vi "Menu.Sequeunce.Execute.vi"(8 "error in (no error)":errorcluster, 9 "Coords":T1, 10 "ItemPath":string, 11 "State Variables":T2={"Aliases.All"=[], "Aliases.Outputs"=[], "UI.Sequence#ofColumns"=0, "SysDef.Path"=path "", "UI.SequenceRef"=refnum, "UI.StepInformationRef"=refnum, "UI.AbortRef"=refnum, "UI.GraphRef"=refnum, "UI.ViewRef"=refnum, "UI.IterationsRef"=refnum, "UI.IterationInformationRef"=refnum, "INI.Settings"={"Build Location"=path "C:/Simple Sequence Editor/SequenceRepo", "LoggingLocation"=path ""}, "NIVS.Workspace Event"=refnum, "UI.SkipChannel"=refnum, "NIVS.Launched?"=FALSE, "UI.DurationChannel"=refnum}) -> (0 "error out":errorcluster, 3 "State Variables out":T2={"Aliases.All"=[], "Aliases.Outputs"=[], "UI.Sequence#ofColumns"=0, "SysDef.Path"=path "", "UI.SequenceRef"=refnum, "UI.StepInformationRef"=refnum, "UI.AbortRef"=refnum, "UI.GraphRef"=refnum, "UI.ViewRef"=refnum, "UI.IterationsRef"=refnum, "UI.IterationInformationRef"=refnum, "INI.Settings"={"Build Location"=path "C:/Simple Sequence Editor/SequenceRepo", "LoggingLocation"=path ""}, "NIVS.Workspace Event"=refnum, "UI.SkipChannel"=refnum, "NIVS.Launched?"=FALSE, "UI.DurationChannel"=refnum})   [LabVIEW 2015, in "Simple Sequence Tools - Editor.lvlib"]
uses:
  Simple Sequence Tools - Editor.lvlib
  Types/Main.StateVariables.ctl
  Shared/Types/Channel.Properties.ctl
  Shared/Types/INI.Settings.ctl
  <vilib>/Utility/miscctls.llb/LVPoint32TypeDef.ctl
  <vilib>/Utility/miscctls.llb/LVBoundsTypeDef.ctl
  Shared/SubVIs/Main.Constants.vi
  Shared/Simple Sequence Tools - Shared.lvlib
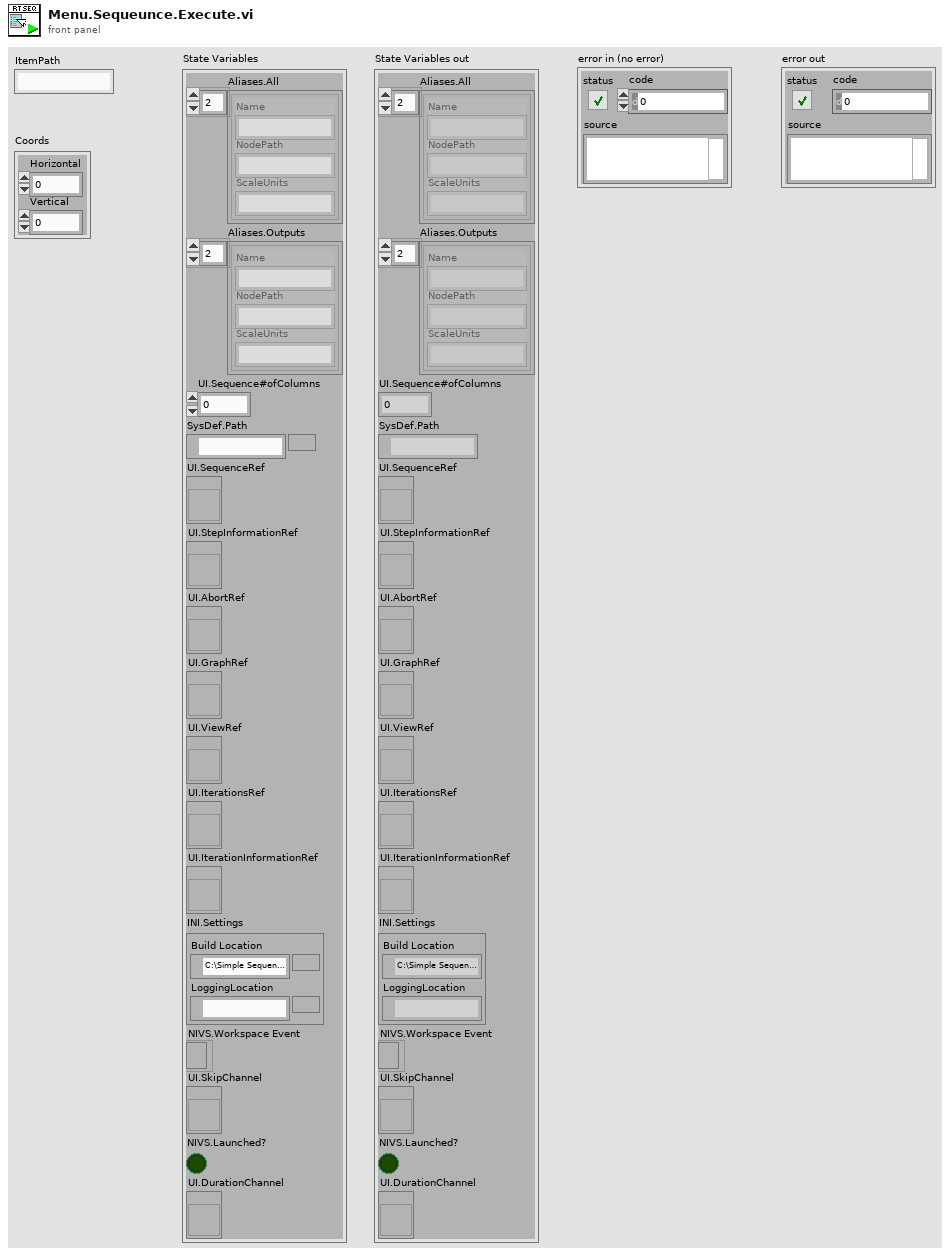
[diagram p1: front panel]
types:
  T1 = typedef "LVPoint32TypeDef.ctl" = cluster{"Horizontal":i32, "Vertical":i32}
  T2 = typedef "Simple Sequence Tools - Editor.lvlib/Main.StateVariables.ctl" = cluster{"Aliases.All":T3[], "Aliases.Outputs":T3[], "UI.Sequence#ofColumns":i32, "SysDef.Path":path, "UI.SequenceRef":refnum<vi>, "UI.StepInformationRef":refnum<vi>, "UI.AbortRef":refnum<vi>, "UI.GraphRef":refnum<vi>, "UI.ViewRef":refnum<vi>, "UI.IterationsRef":refnum<vi>, "UI.IterationInformationRef":refnum<vi>, "INI.Settings":T4, "NIVS.Workspace Event":refnum<event-registration>, "UI.SkipChannel":refnum<vi>, "NIVS.Launched?":bool, "UI.DurationChannel":refnum<vi>}
  T3 = typedef "Simple Sequence Tools - Shared.lvlib/Channel.Properties.ctl" = cluster{"Name":string, "NodePath":string, "ScaleUnits":string}
  T4 = typedef "Simple Sequence Tools - Shared.lvlib/INI.Settings.ctl" = cluster{"Build Location":path, "LoggingLocation":path}
  T5 = typedef "LVRowAndColumnTypeDef.ctl" = cluster{"Row":i32, "Column":i32}
  T6 = typedef "LVBoundsTypeDef.ctl" = cluster{"Width":u32, "Height":u32}
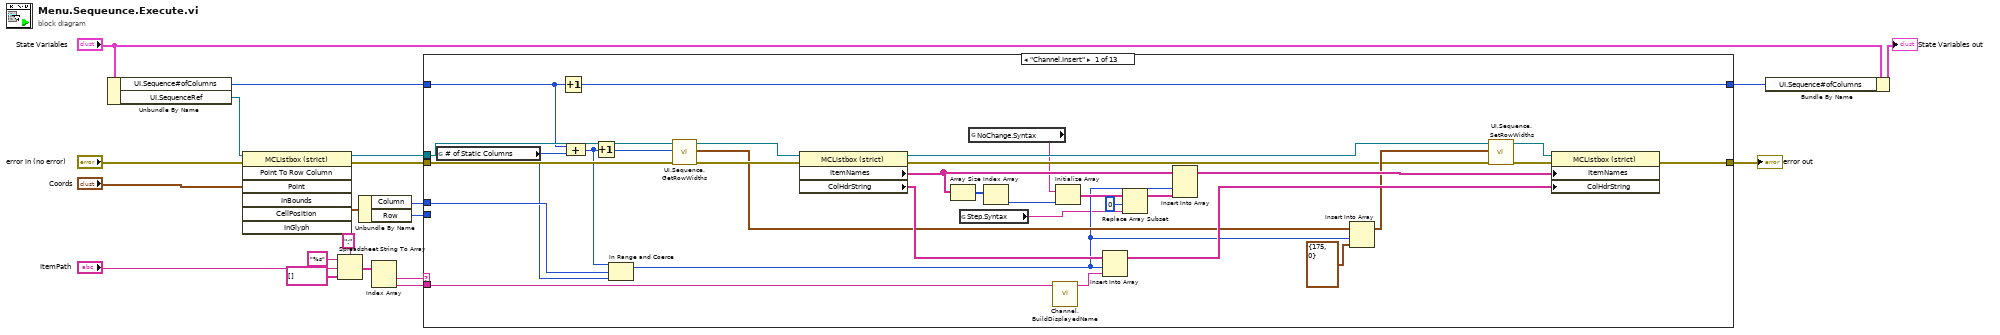
[diagram p0: block diagram]
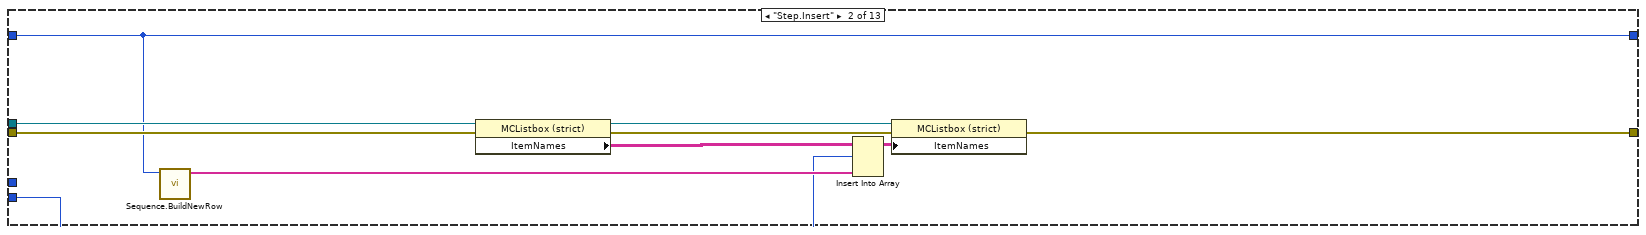
[diagram p2: hidden frame]
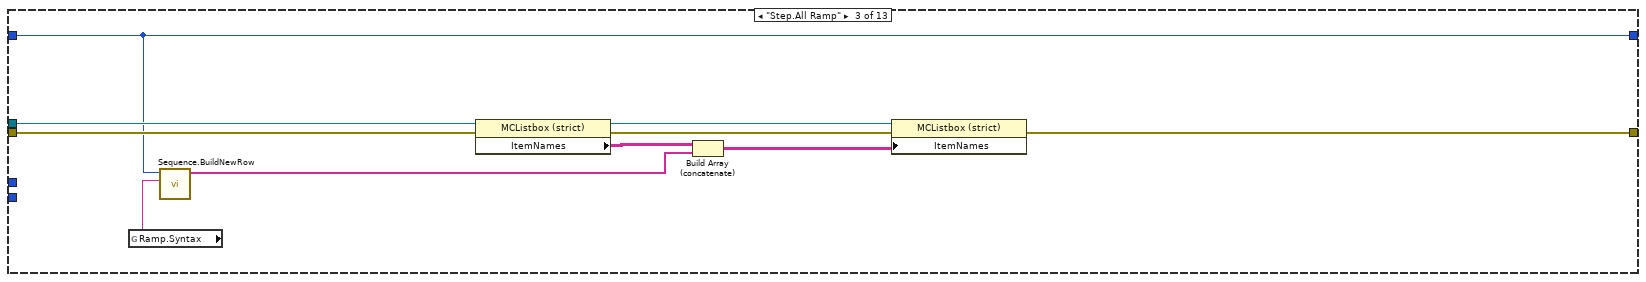
[diagram p3: hidden frame]
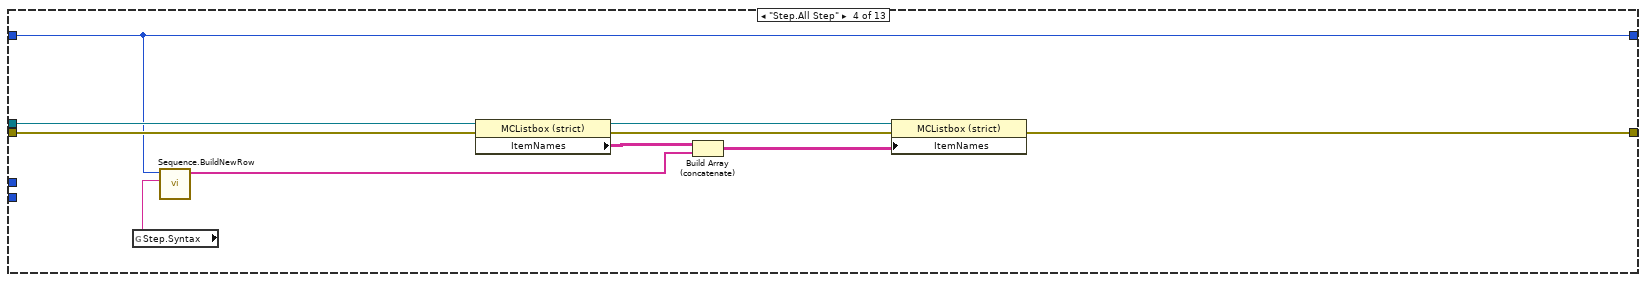
[diagram p4: hidden frame]
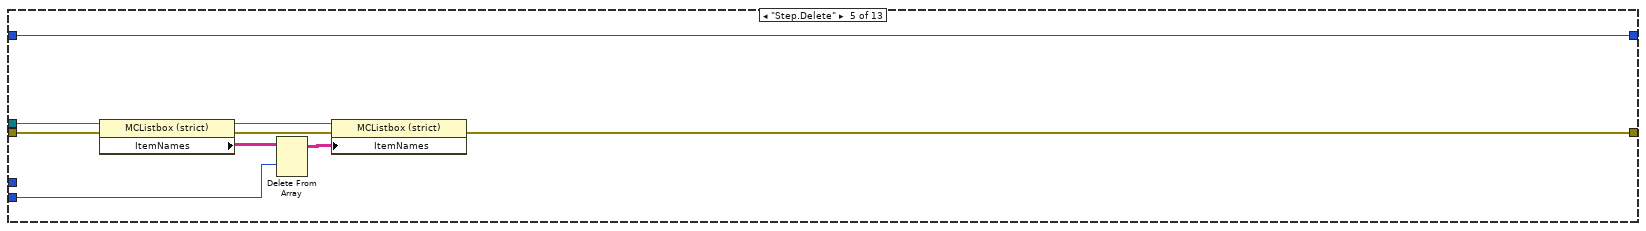
[diagram p5: hidden frame]
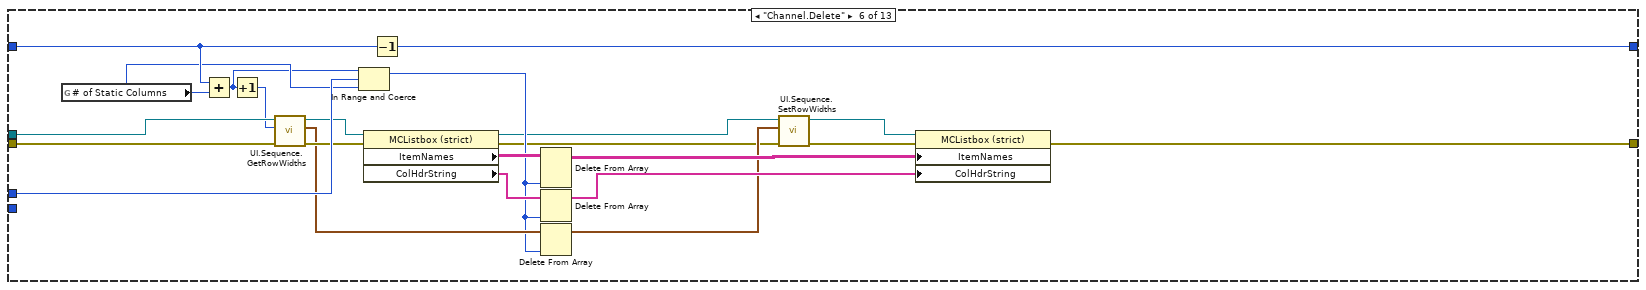
[diagram p6: hidden frame]
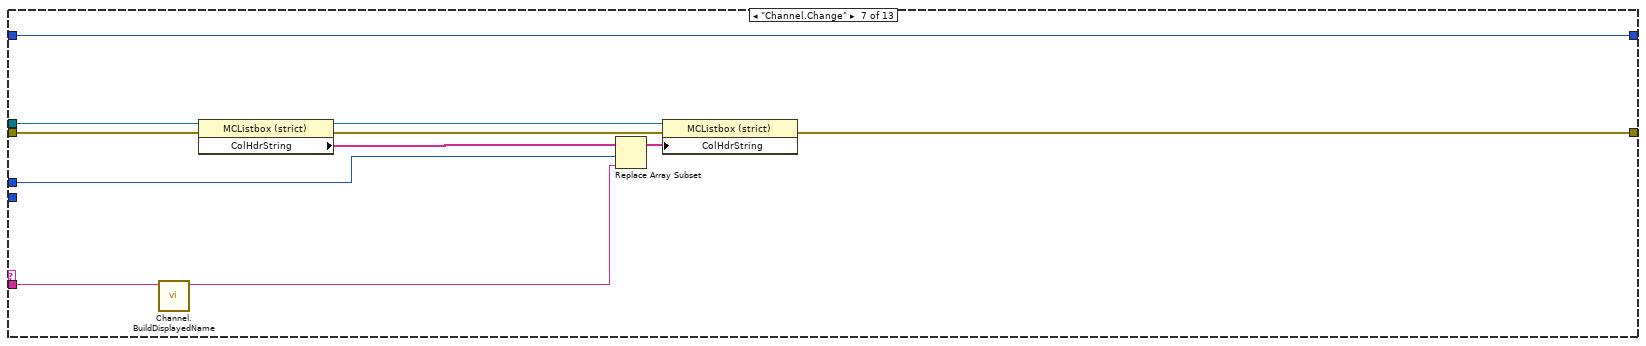
[diagram p7: hidden frame]
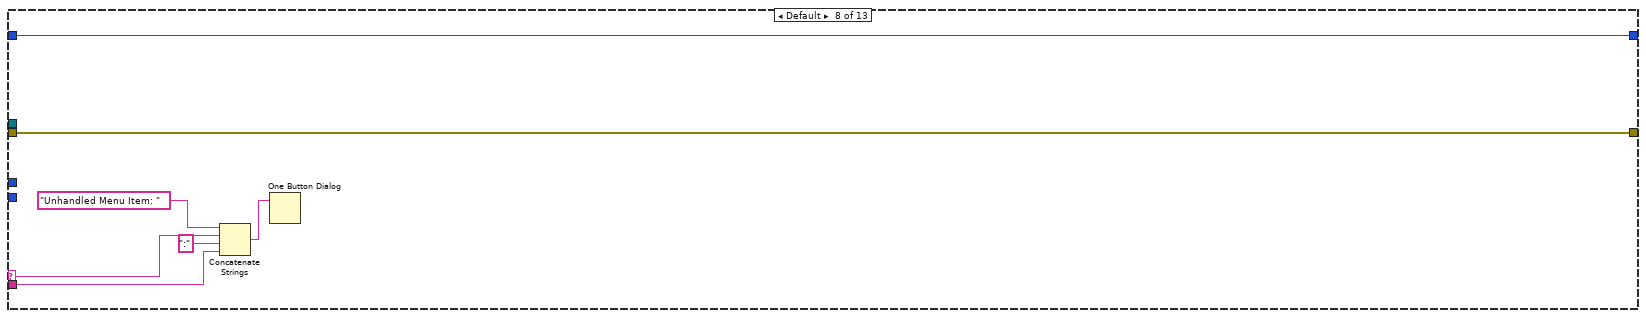
[diagram p8: hidden frame]
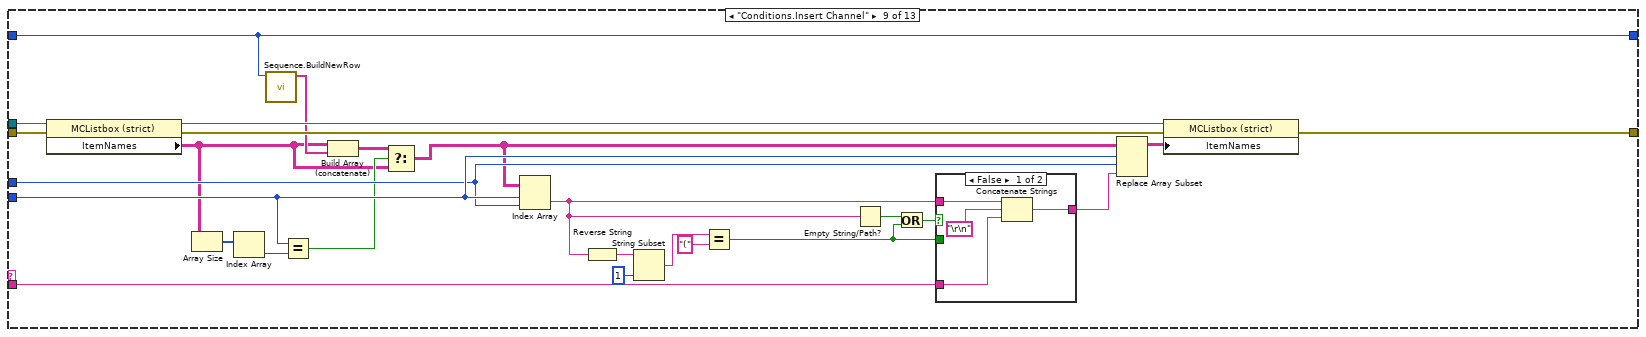
[diagram p9: hidden frame]
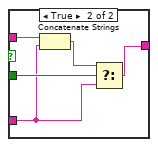
[diagram p10: hidden frame]
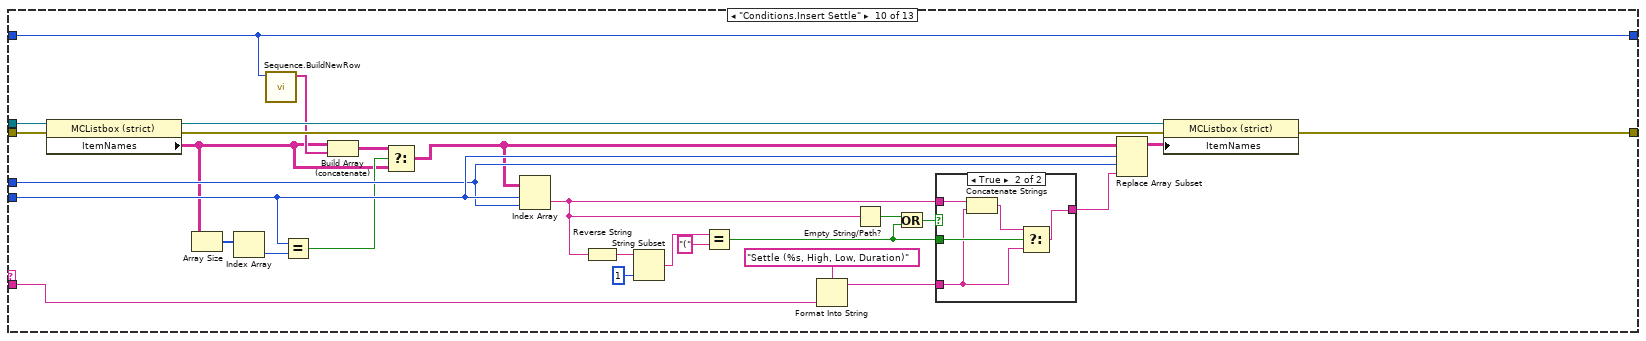
[diagram p11: hidden frame]
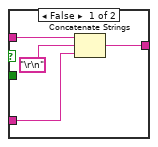
[diagram p12: hidden frame]
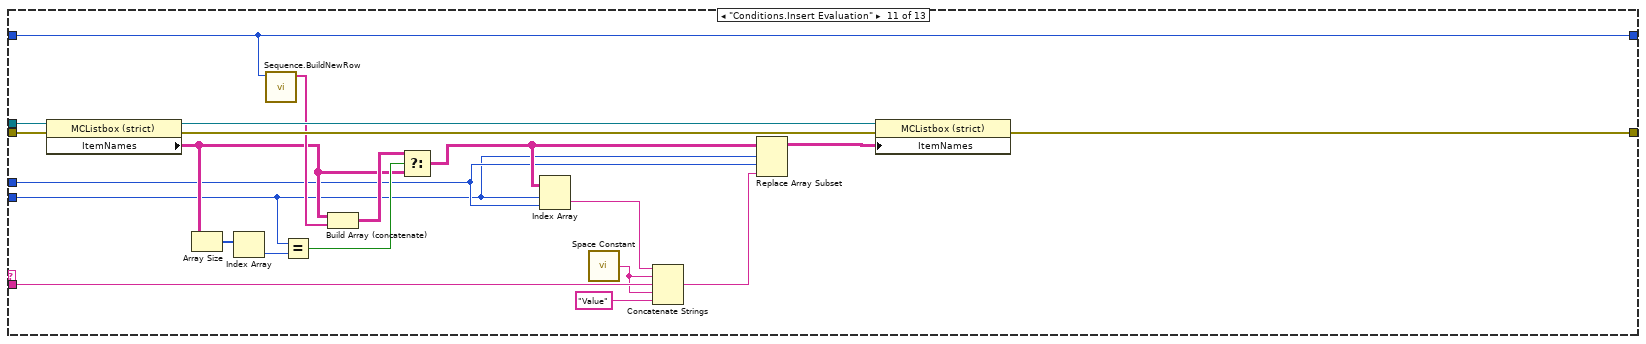
[diagram p13: hidden frame]
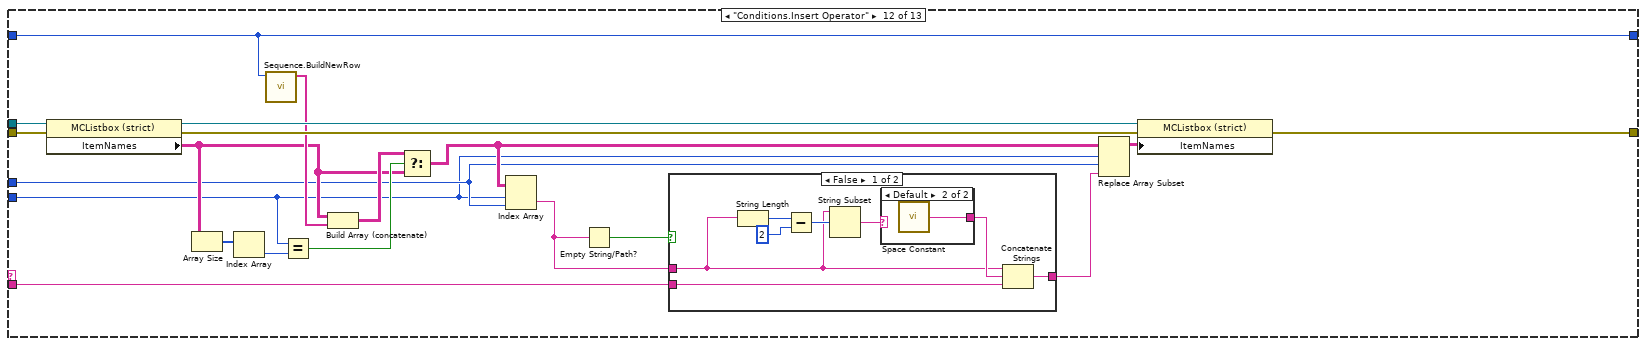
[diagram p14: hidden frame]
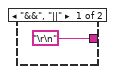
[diagram p15: hidden frame]
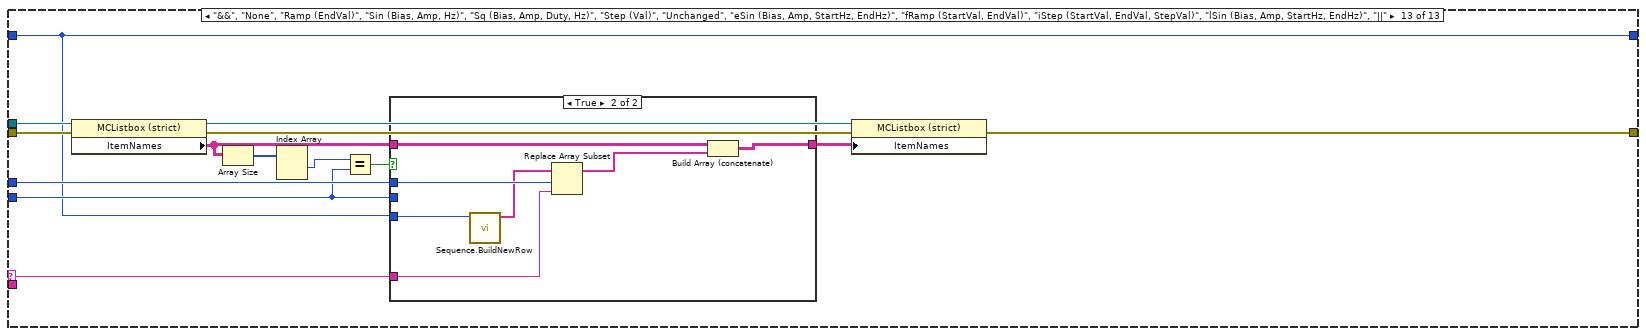
[diagram p17: hidden frame]
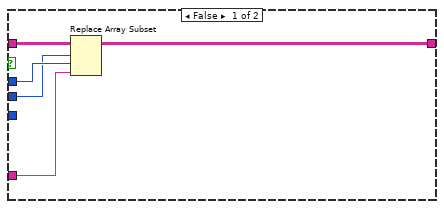
[diagram p18: hidden frame]
diagram:
  n1 = Unbundle By Name("State Variables") -> ("UI.Sequence#ofColumns"=w11:i32, "UI.SequenceRef"=w8:refnum<vi>)
  n2 = invoke class="MCListbox (strict)" method="Point To Row Column"(reference=w8, error in="error in (no error)", "Point"="Coords") -> (reference out=w13:refnum<vi>, error out=w14:errorcluster, "CellPosition"=w10:T5)  [unwired: 4 in, 4 out]
  n3 = Spreadsheet String To Array(delimiter (Tab)=":", format string="%s", spreadsheet string="ItemPath", array type (2D Dbl)=string[] []) -> (array=w6:string[])
  n4 = Unbundle By Name(w10) -> ("Column"=w12:i32, "Row"=w1:i32)
  n5 = Index Array(array=w6) -> (element #1=w7:string, element #2=w15:string)  [unwired: 2 in]
  n6 = case shown="\"Channel.Insert\"" w7 {
    selector: w7 -> [_ _ _ _ _ _ _ w129 _ _ _ _ w258]
    tunnel: w11 -> [w36 w53 w65 w75 w83 w100 w124 w131 w148 w186 w217 w237 w256]
    tunnel: w12 -> [w52 _ _ _ _ w113 w117 _ w142 w180 w207 w228 w264]
    tunnel: w13 -> [w38 w58 w68 w78 w87 w105 w118 _ w157 w194 w224 w244 w268]
    tunnel: w14 -> [w40 w59 w69 w79 w88 w107 w119 w130 w156 w193 w223 w243 w269]
    tunnel: w15 -> [w42 _ _ _ _ _ w115 w127 w152 w167 w219 w239 _]
    tunnel: [w24 w60 w70 w80 w89 w94 w116 w130 w154 w191 w221 w241 w257] -> w17
    tunnel: [w35 w53 w65 w75 w83 w112 w124 w131 w148 w186 w217 w237 w256] -> w20
    tunnel: w1 -> [_ w54 _ _ w84 _ _ _ w145 w183 w206 w227 w260]
    frame "Channel.Insert" {
      n7 = global read "Main.Constants.vi" "# of Static Columns"() -> (w22:u32)
      n8 = Increment(x=w36) -> (x+1=w35:i32)
      n9 = Compound Arithmetic op=ADD(w36, w22) -> (w21:u32)
      n10 = Increment(x=w21) -> (x+1=w30:u32)
      n11 = In Range and Coerce(upper limit=w21, x=w52, lower limit=w22) -> (coerced(x)=w32:u32)  [unwired: 1 out]
      n12 = call "UI.Sequence.GetRowWidths.vi"("error in (no error)"=w40, "Numeric"=w30, "UI.SequenceRef"=w38) -> ("error out"=w39:errorcluster, "Array"=w33:T6[], "UI.SequenceRef"=w37:refnum<vi>)  [unwired: 6 in]
      n13 = property class="MCListbox (strict)"(reference=w37, error in=w39) -> (reference out=w25:refnum<vi>, error out=w28:errorcluster, "ItemNames"=w50:string[][], "ColHdrString"=w45:string[])
      n14 = Array Size(array=w50) -> (size(s)=w51:i32[])
      n15 = global read "Main.Constants.vi" "Step.Syntax"() -> (w29:string)
      n16 = global read "Main.Constants.vi" "NoChange.Syntax"() -> (w23:string)
      n17 = Index Array(array=w51) -> (element=w49:i32)  [unwired: 1 in]
      n18 = call "Channel.BuildDisplayedName.vi"("Path"=w42) -> ("Formated Path"=w41:string)  [unwired: 10 in]
      n19 = Initialize Array(w23, w49) -> (w48:string[])
      n20 = Insert Into Array(array=w45, index=w32, new element=w41) -> (w46:string[])
      n21 = Replace Array Subset(array=w48, new element=w29, index=0) -> (w44:string[])
      n22 = Insert Into Array(array=w50, index (col)=w32, new element=w44) -> (w47:string[][])  [unwired: 1 in]
      n23 = Insert Into Array(array=w33, index=w32, new element=T6 {"Width"=175, "Height"=0} ("new element/subarray")) -> (w34:T6[])
      n24 = call "UI.Sequence.SetRowWidths.vi"("error in (no error)"=w28, "CellSize"=w34, "UI.SequenceRef"=w25) -> ("error out"=w27:errorcluster, "UI.SequenceRef"=w26:refnum<vi>)  [unwired: 7 in]
      n25 = property class="MCListbox (strict)"(reference=w26, error in=w27, "ItemNames"=w47, "ColHdrString"=w46) -> (error out=w24:errorcluster)  [unwired: 1 out]
    }
    frame "Step.Insert" {
      n26 = call "Sequence.BuildNewRow.vi"("UI.Sequence#ofColumns"=w53) -> ("New Array"=w57:string[])  [unwired: 10 in]
      n27 = property class="MCListbox (strict)"(reference=w58, error in=w59) -> (reference out=w55:refnum<vi>, error out=w56:errorcluster, "ItemNames"=w62:string[][])
      n28 = Insert Into Array(array=w62, index (row)=w54, new element=w57) -> (w61:string[][])  [unwired: 1 in]
      n29 = property class="MCListbox (strict)"(reference=w55, error in=w56, "ItemNames"=w61) -> (error out=w60:errorcluster)  [unwired: 1 out]
    }
    frame "Step.All Ramp" {
      n30 = global read "Main.Constants.vi" "Ramp.Syntax"() -> (w64:string)
      n31 = call "Sequence.BuildNewRow.vi"("Syntax"=w64, "UI.Sequence#ofColumns"=w65) -> ("New Array"=w63:string[])  [unwired: 9 in]
      n32 = property class="MCListbox (strict)"(reference=w68, error in=w69) -> (reference out=w66:refnum<vi>, error out=w67:errorcluster, "ItemNames"=w72:string[][])
      n33 = Build Array (concatenate)(w72, w63) -> (w71:string[][])
      n34 = property class="MCListbox (strict)"(reference=w66, error in=w67, "ItemNames"=w71) -> (error out=w70:errorcluster)  [unwired: 1 out]
    }
    frame "Step.All Step" {
      n35 = global read "Main.Constants.vi" "Step.Syntax"() -> (w74:string)
      n36 = call "Sequence.BuildNewRow.vi"("Syntax"=w74, "UI.Sequence#ofColumns"=w75) -> ("New Array"=w73:string[])  [unwired: 9 in]
      n37 = property class="MCListbox (strict)"(reference=w78, error in=w79) -> (reference out=w76:refnum<vi>, error out=w77:errorcluster, "ItemNames"=w82:string[][])
      n38 = Build Array (concatenate)(w82, w73) -> (w81:string[][])
      n39 = property class="MCListbox (strict)"(reference=w76, error in=w77, "ItemNames"=w81) -> (error out=w80:errorcluster)  [unwired: 1 out]
    }
    frame "Step.Delete" {
      n40 = property class="MCListbox (strict)"(reference=w87, error in=w88) -> (reference out=w85:refnum<vi>, error out=w86:errorcluster, "ItemNames"=w91:string[][])
      n41 = Delete From Array(array=w91, index (row)=w84) -> (array with subset deleted=w90:string[][])  [unwired: 2 in, 1 out]
      n42 = property class="MCListbox (strict)"(reference=w85, error in=w86, "ItemNames"=w90) -> (error out=w89:errorcluster)  [unwired: 1 out]
    }
    frame "Channel.Delete" {
      n43 = global read "Main.Constants.vi" "# of Static Columns"() -> (w93:u32)
      n44 = Add(x=w100, y=w93) -> (x+y=w92:u32)
      n45 = Increment(x=w92) -> (x+1=w99:u32)
      n46 = call "UI.Sequence.GetRowWidths.vi"("error in (no error)"=w107, "Numeric"=w99, "UI.SequenceRef"=w105) -> ("error out"=w106:errorcluster, "Array"=w103:T6[], "UI.SequenceRef"=w104:refnum<vi>)  [unwired: 6 in]
      n47 = In Range and Coerce(upper limit=w92, x=w113, lower limit=w93) -> (coerced(x)=w102:u32)  [unwired: 1 out]
      n48 = property class="MCListbox (strict)"(reference=w104, error in=w106) -> (reference out=w95:refnum<vi>, error out=w98:errorcluster, "ItemNames"=w111:string[][], "ColHdrString"=w108:string[])
      n49 = Decrement(x=w100) -> (x-1=w112:i32)
      n50 = Delete From Array(array=w111, index (col)=w102) -> (array with subset deleted=w110:string[][])  [unwired: 2 in, 1 out]
      n51 = Delete From Array(array=w108, index=w102) -> (array with subset deleted=w109:string[])  [unwired: 1 in, 1 out]
      n52 = Delete From Array(array=w103, index=w102) -> (array with subset deleted=w101:T6[])  [unwired: 1 in, 1 out]
      n53 = call "UI.Sequence.SetRowWidths.vi"("error in (no error)"=w98, "CellSize"=w101, "UI.SequenceRef"=w95) -> ("error out"=w97:errorcluster, "UI.SequenceRef"=w96:refnum<vi>)  [unwired: 7 in]
      n54 = property class="MCListbox (strict)"(reference=w96, error in=w97, "ItemNames"=w110, "ColHdrString"=w109) -> (error out=w94:errorcluster)  [unwired: 1 out]
    }
    frame "Channel.Change" {
      n55 = call "Channel.BuildDisplayedName.vi"("Path"=w115) -> ("Formated Path"=w114:string)  [unwired: 10 in]
      n56 = property class="MCListbox (strict)"(reference=w118, error in=w119) -> (reference out=w123:refnum<vi>, error out=w122:errorcluster, "ColHdrString"=w120:string[])
      n57 = Replace Array Subset(array=w120, new element=w114, index=w117) -> (w121:string[])
      n58 = property class="MCListbox (strict)"(reference=w123, error in=w122, "ColHdrString"=w121) -> (error out=w116:errorcluster)  [unwired: 1 out]
    }
    frame Default {
      n59 = Concatenate Strings("Unhandled Menu Item: " ("message"), w129, ":" ("string"), w127) -> (w125:string)
      n60 = One Button Dialog(message=w125) -> ()  [unwired: 1 in, 1 out]
    }
    frame "Conditions.Insert Channel" {
      n61 = property class="MCListbox (strict)"(reference=w157, error in=w156) -> (reference out=w153:refnum<vi>, error out=w155:errorcluster, "ItemNames"=w140:string[][])
      n62 = Array Size(array=w140) -> (size(s)=w147:i32[])
      n63 = Index Array(array=w147) -> (element=w146:i32)  [unwired: 1 in]
      n64 = call "Sequence.BuildNewRow.vi"("UI.Sequence#ofColumns"=w148) -> ("New Array"=w144:string[])  [unwired: 10 in]
      n65 = Equal?(x=w145, y=w146) -> (x = y?=w141:bool)
      n66 = Build Array (concatenate)(w140, w144) -> (w143:string[][])
      n67 = Select(t=w143, s=w141, f=w140) -> (s? t:f=w137:string[][])
      n68 = Index Array(array=w137, index (row)=w145, index (col)=w142) -> (element=w133:string)
      n69 = Reverse String(1:w133) -> (0:w135:string)
      n70 = String Subset(string=w135, length (rest)=1 ("length (rest)")) -> (substring=w132:string)  [unwired: 1 in]
      n71 = Equal?(x=w132, y="(") -> (x = y?=w136:bool)
      n72 = Empty String/Path?(string/path=w133) -> (empty?=w151:bool)
      n73 = Or(x=w151, y=w136) -> (x .or. y?=w138:bool)
      n74 = case shown="False" w138 {
        tunnel: w133 -> [w161 w165]
        tunnel: w152 -> [w160 w164]
        tunnel: [w158 w163] -> w150
        tunnel: w136 -> [_ w166]
        frame False {
          n75 = Concatenate Strings(w161, "\r\n", w160) -> (w158:string)
        }
        frame True {
          n76 = Concatenate Strings(w165, w164) -> (w162:string)
          n77 = Select(t=w162, s=w166, f=w164) -> (s? t:f=w163:string)
        }
      }
      n78 = Replace Array Subset(array=w137, new element=w150, index (row)=w145, index (col)=w142) -> (w149:string[][])
      n79 = property class="MCListbox (strict)"(reference=w153, error in=w155, "ItemNames"=w149) -> (error out=w154:errorcluster)  [unwired: 1 out]
    }
    frame "Conditions.Insert Settle" {
      n80 = property class="MCListbox (strict)"(reference=w194, error in=w193) -> (reference out=w190:refnum<vi>, error out=w192:errorcluster, "ItemNames"=w178:string[][])
      n81 = Array Size(array=w178) -> (size(s)=w185:i32[])
      n82 = Index Array(array=w185) -> (element=w184:i32)  [unwired: 1 in]
      n83 = call "Sequence.BuildNewRow.vi"("UI.Sequence#ofColumns"=w186) -> ("New Array"=w182:string[])  [unwired: 10 in]
      n84 = Equal?(x=w183, y=w184) -> (x = y?=w179:bool)
      n85 = Build Array (concatenate)(w178, w182) -> (w181:string[][])
      n86 = Select(t=w181, s=w179, f=w178) -> (s? t:f=w175:string[][])
      n87 = Index Array(array=w175, index (row)=w183, index (col)=w180) -> (element=w171:string)
      n88 = Reverse String(1:w171) -> (0:w173:string)
      n89 = String Subset(string=w173, length (rest)=1 ("length (rest)")) -> (substring=w170:string)  [unwired: 1 in]
      n90 = Equal?(x=w170, y="(") -> (x = y?=w174:bool)
      n91 = Format Into String(format string="Settle (%s, High, Low, Duration)", w167) -> (resulting string=w169:string)  [unwired: 2 in, 1 out]
      n92 = Empty String/Path?(string/path=w171) -> (empty?=w189:bool)
      n93 = Or(x=w189, y=w174) -> (x .or. y?=w176:bool)
      n94 = case shown="True" w176 {
        tunnel: w171 -> [w198 w202]
        tunnel: w169 -> [w197 w201]
        tunnel: [w195 w200] -> w188
        tunnel: w174 -> [_ w203]
        frame False {
          n95 = Concatenate Strings(w198, "\r\n", w197) -> (w195:string)
        }
        frame True {
          n96 = Concatenate Strings(w202, w201) -> (w199:string)
          n97 = Select(t=w199, s=w203, f=w201) -> (s? t:f=w200:string)
        }
      }
      n98 = Replace Array Subset(array=w175, new element=w188, index (row)=w183, index (col)=w180) -> (w187:string[][])
      n99 = property class="MCListbox (strict)"(reference=w190, error in=w192, "ItemNames"=w187) -> (error out=w191:errorcluster)  [unwired: 1 out]
    }
    frame "Conditions.Insert Evaluation" {
      n100 = property class="MCListbox (strict)"(reference=w224, error in=w223) -> (reference out=w220:refnum<vi>, error out=w222:errorcluster, "ItemNames"=w211:string[][])
      n101 = Array Size(array=w211) -> (size(s)=w216:i32[])
      n102 = Index Array(array=w216) -> (element=w215:i32)  [unwired: 1 in]
      n103 = call "Sequence.BuildNewRow.vi"("UI.Sequence#ofColumns"=w217) -> ("New Array"=w214:string[])  [unwired: 10 in]
      n104 = Equal?(x=w206, y=w215) -> (x = y?=w212:bool)
      n105 = Build Array (concatenate)(w211, w214) -> (w213:string[][])
      n106 = Select(t=w213, s=w212, f=w211) -> (s? t:f=w208:string[][])
      n107 = Index Array(array=w208, index (row)=w206, index (col)=w207) -> (element=w204:string)
      n108 = call <vilib>:"Space Constant.vi"() -> ("String"=w205:string)
      n109 = Concatenate Strings(w204, w205, w219, w205, "Value" ("string")) -> (w210:string)
      n110 = Replace Array Subset(array=w208, new element=w210, index (row)=w206, index (col)=w207) -> (w218:string[][])
      n111 = property class="MCListbox (strict)"(reference=w220, error in=w222, "ItemNames"=w218) -> (error out=w221:errorcluster)  [unwired: 1 out]
    }
    frame "Conditions.Insert Operator" {
      n112 = property class="MCListbox (strict)"(reference=w244, error in=w243) -> (reference out=w240:refnum<vi>, error out=w242:errorcluster, "ItemNames"=w231:string[][])
      n113 = Array Size(array=w231) -> (size(s)=w236:i32[])
      n114 = Index Array(array=w236) -> (element=w235:i32)  [unwired: 1 in]
      n115 = call "Sequence.BuildNewRow.vi"("UI.Sequence#ofColumns"=w237) -> ("New Array"=w234:string[])  [unwired: 10 in]
      n116 = Equal?(x=w227, y=w235) -> (x = y?=w232:bool)
      n117 = Build Array (concatenate)(w231, w234) -> (w233:string[][])
      n118 = Select(t=w233, s=w232, f=w231) -> (s? t:f=w229:string[][])
      n119 = Index Array(array=w229, index (row)=w227, index (col)=w228) -> (element=w226:string)
      n120 = Empty String/Path?(string/path=w226) -> (empty?=w225:bool)
      n121 = case shown="False" w225 {
        tunnel: w239 -> [w252 w255]
        tunnel: [w251 w255] -> w230
        tunnel: w226 -> [w245 _]
        frame False {
          n122 = String Length(string=w245) -> (length=w250:i32)
          n123 = Subtract(x=w250, y=2) -> (x-y=w249:i32)
          n124 = String Subset(string=w245, offset (0)=w249) -> (substring=w247:string)  [unwired: 1 in]
          n125 = case shown="Default" w247 {
            tunnel: ["\r\n" w254] -> w246
            frame "&&", "||" {
            }
            frame Default {
              n126 = call <vilib>:"Space Constant.vi"() -> ("String"=w254:string)
            }
          }
          n127 = Concatenate Strings(w245, w246, w252) -> (w251:string)
        }
        frame True {
        }
      }
      n128 = Replace Array Subset(array=w229, new element=w230, index (row)=w227, index (col)=w228) -> (w238:string[][])
      n129 = property class="MCListbox (strict)"(reference=w240, error in=w242, "ItemNames"=w238) -> (error out=w241:errorcluster)  [unwired: 1 out]
    }
    frame "&&", "None", "Ramp (EndVal)", "Sin (Bias, Amp, Hz)", "Sq (Bias, Amp, Duty, Hz)", "Step (Val)", "Unchanged", "eSin (Bias, Amp, StartHz, EndHz)", "fRamp (StartVal, EndVal)", "iStep (StartVal, EndVal, StepVal)", "lSin (Bias, Amp, StartHz, EndHz)", "||" {
      n130 = property class="MCListbox (strict)"(reference=w268, error in=w269) -> (reference out=w266:refnum<vi>, error out=w267:errorcluster, "ItemNames"=w263:string[][])
      n131 = Array Size(array=w263) -> (size(s)=w262:i32[])
      n132 = Index Array(array=w262) -> (element #1=w261:i32)  [unwired: 2 in, 1 out]
      n133 = Equal?(x=w261, y=w260) -> (x = y?=w259:bool)
      n134 = case shown="True" w259 {
        tunnel: [w274 w280] -> w265
        tunnel: w264 -> [w273 w279]
        tunnel: w263 -> [w272 w281]
        tunnel: w260 -> [w271 _]
        tunnel: w256 -> [_ w276]
        tunnel: w258 -> [w270 w278]
        frame False {
          n135 = Replace Array Subset(array=w272, new element=w270, index (row)=w271, index (col)=w273) -> (w274:string[][])
        }
        frame True {
          n136 = call "Sequence.BuildNewRow.vi"("UI.Sequence#ofColumns"=w276) -> ("New Array"=w275:string[])  [unwired: 10 in]
          n137 = Replace Array Subset(array=w275, new element=w278, index=w279) -> (w277:string[])
          n138 = Build Array (concatenate)(w281, w277) -> (w280:string[][])
        }
      }
      n139 = property class="MCListbox (strict)"(reference=w266, error in=w267, "ItemNames"=w265) -> (error out=w257:errorcluster)  [unwired: 1 out]
    }
  }
  "error out" <- w17
  n140 = Bundle By Name(cluster="State Variables", "UI.Sequence#ofColumns"=w20) -> (→"State Variables out":T2)
